vi "Visu acqui.vi"() -> ()   [LabVIEW 2022 SP3]
uses:
  Enum/Enum 7.ctl
  Variables globales/Variable glob generale.vi
  Variables globales/Variable globale compteurs.vi
  Variables globales/Variable glob Keller.vi
  Variables globales/Variable glob Pt.vi
  Variables globales/Variable glob Leybold.vi
  Variables globales/Variable glob Edwards.vi
  Variables globales/Variable glob Th.vi
  Variables globales/Variables glob EUROTHERM.vi
  Variables globales/Variable glob alertes pressions.vi
  Variables globales/Variable glob alertes min-max temperatures.vi
  Variables globales/Variable glob alertes ecart temperatures.vi
  Variables globales/Variable glob alertes Keller.vi
  Variables globales/Variable glob alertes Compteurs.vi
  <vilib>/Utility/config.llb/Write Key (String).vi
  <vilib>/Utility/config.llb/NI_LVConfig.lvlib
panel:
  in  "Y1/Y2":cluster{"Booléen":bool}[][](array[cluster]) caption="Y1    Y2"
  out "Alerte Compteurs":bool caption="Compteurs"
  in  "voir compteurs":bool caption="Valeurs compteurs"
  in  "Unités par":u16(ring) items=["seconde", "minute", "heure"]
  out "Pente":dbl format="%#.2g"
  in  "Capteur":u16(ring) items=[" keller1", "Compteur Sortie BLN2", "Débit Sortie BLN2"]
  in  "Calcul Pente":bool
  in  "voir alertes":bool caption="Définitions Alertes"
  out "nb capt":i32
  out "Noms visu":string[](array[string])
  out "Cuve":string
  out "Dossier distant":path
  out "référence en sortie":refnum<vi>
  out "SORTIE VISU":bool
  in  "Tout Y2":bool
  out "commentaire":string
  out "Dossier de sauvegarde":path
  in  "Tout Y1":bool
  in  "Tout OFF":bool
  out "Chemin du fichier local":path
  in  "Couleurs":u32[](array[colorbox])
  out "Alerte écart temp":bool caption="écarts températures"
  in  "Y2 log":bool caption="Y2 lin"
  in  "Y1 log":bool caption="Y1 lin"
  out "Alerte Keller":bool caption="Keller"
  out "Alerte min/max temp":bool caption="min/max températures"
  out "Données":string[](array[string])
  out "Alerte vide":bool caption="Vide"
  in  "grille Y2":bool
  in  "grille Y1":bool
  out "Courbe":cluster{dbl[], dbl[]}[](graph)
  in  "Echelles des Axes":bool=TRUE
  in  "SORTIR VISU":bool
  # "VISUALISATION ACQUISITIONS\ntempératures et pressions EN COURS"
  # "Ce logiciel et les informations qu'il contient, sont la propriété de l’IAS et ne peuvent être diffusés sans l’autorisation de la Station d’étalonnage"
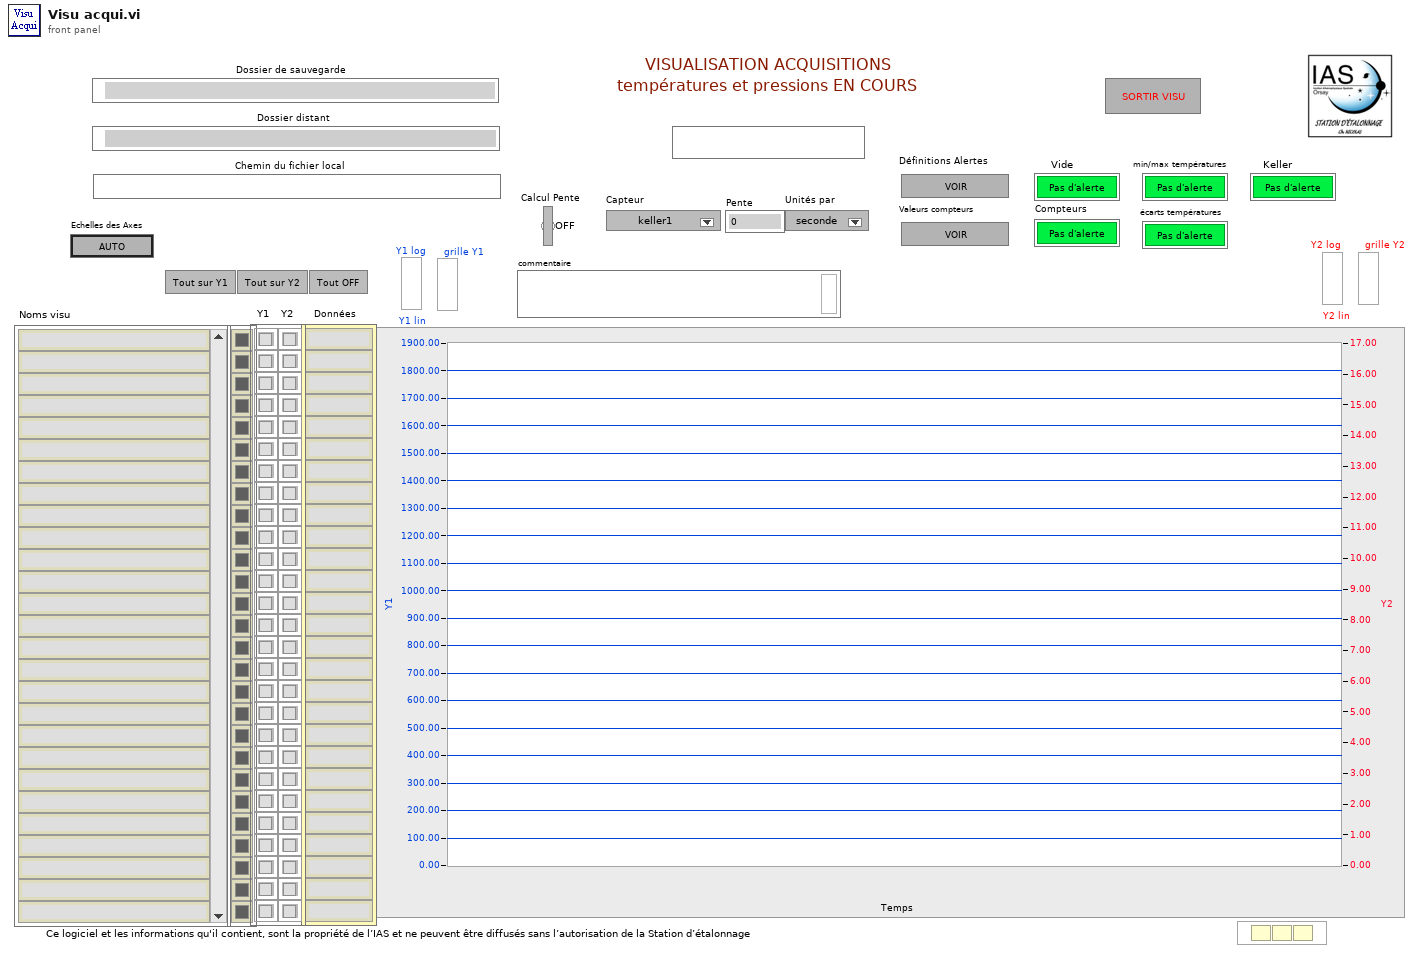
[diagram p1: front panel]
types:
  T1 = typedef "Enum 7.ctl" = enum16{"init", "choix", "init graph", "visu", "choix 2", "fin"}
  T2 = enum32{"Invalid", "Standard", "Closed", "Hidden", "Minimized", "Maximized"}
  T3 = cluster{"Noms voies select acqui 1COM":string[]}[]
  T4 = cluster{"Nom tache compteurs":refnum<k21>, "Noms des compteurs":string[], "Selection":bool[], "Init compteurs":dbl[], "Noms compteurs selectionnes":string[]}
  T5 = cluster{"Nom tache Pt":refnum<k21>, "Noms des Pt":string[], "Nb Pt":i16, "Selection Pt":bool[], "Nom Pt selectionnees":string[]}[]
  T6 = cluster{"Nom tache Th":refnum<k21>, "Noms des Th":string[], "Nb Th":i16, "Selection Th":bool[], "Nom Th selectionnes":string[]}[]
  T7 = cluster{"Alerte temp min/max":bool, "température max":dbl, "température min":dbl, "Défaut min/max temp":bool, "Indices à controler":i16[], "N°":u16}[]
  T8 = cluster{"Indices a controler":i16[], "Defaut":bool, "ecart temp":dbl, "Alerte":bool, ">?":bool, "N°":u16}[]
  T9 = cluster{"Alerte":bool, "valeur alerte":dbl, "Défaut":bool, "Indices à controler":i16[], "N°":u16}[]
  T10 = cluster{"Alerte":bool, "valeur ":dbl, "Défaut":bool, "Indices controler":i16[], "N°":u16}[]
  T11 = cluster{"Alerte Keller":bool, "valeur alerte Keller":dbl, "Défaut Keller":bool, "Indices Keller à controler":i16[], "N°":u16}[]
  T12 = typedef "NI_LVConfig.lvlib/Config Data RefNum.ctl" = refnum<k1>
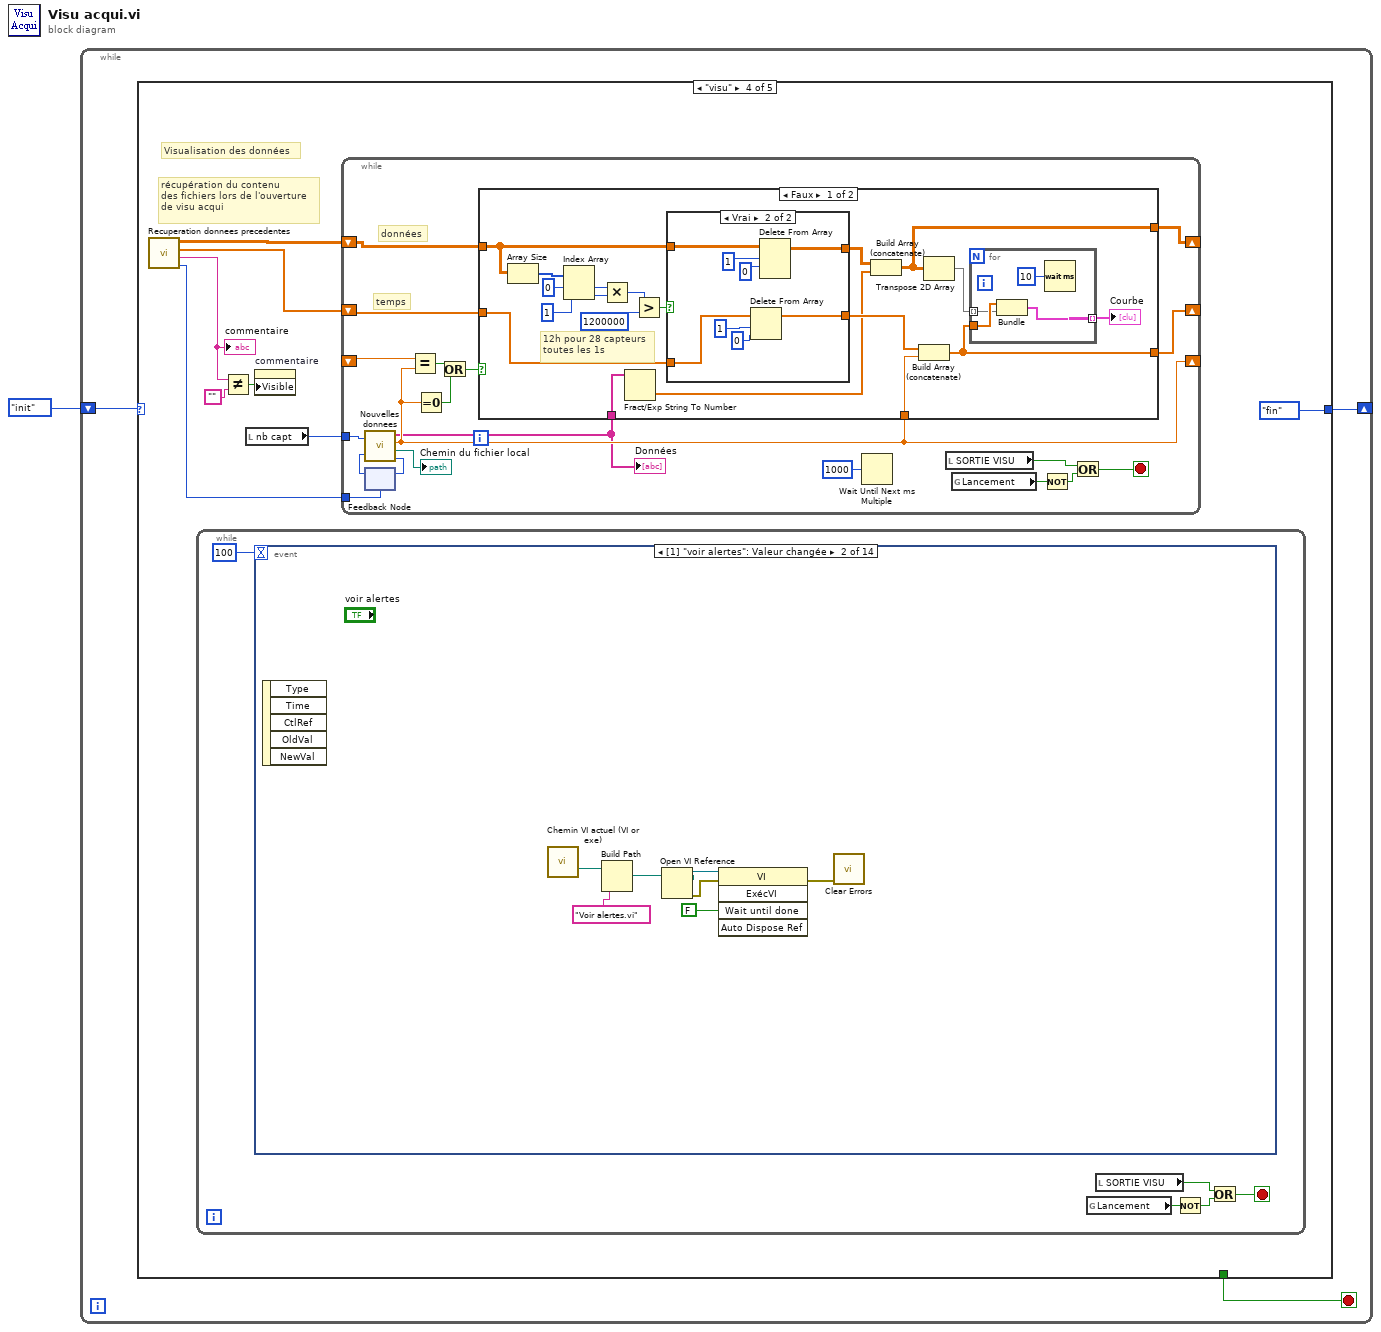
[diagram p0: block diagram]
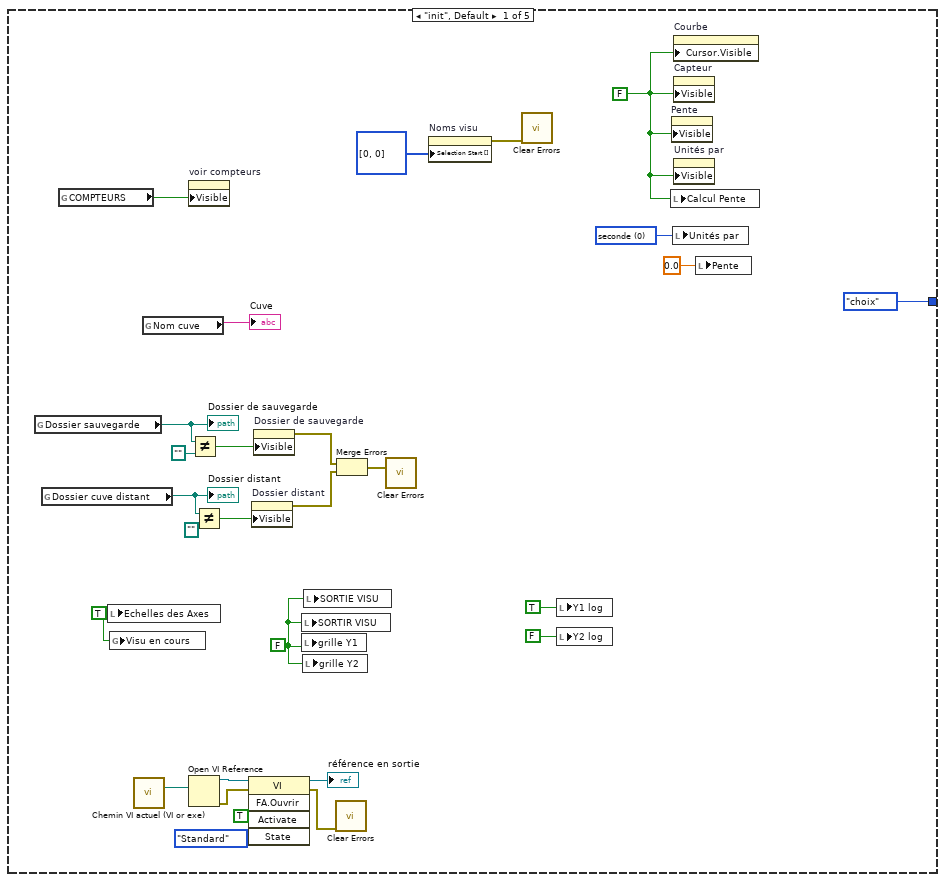
[diagram p2: hidden frame]
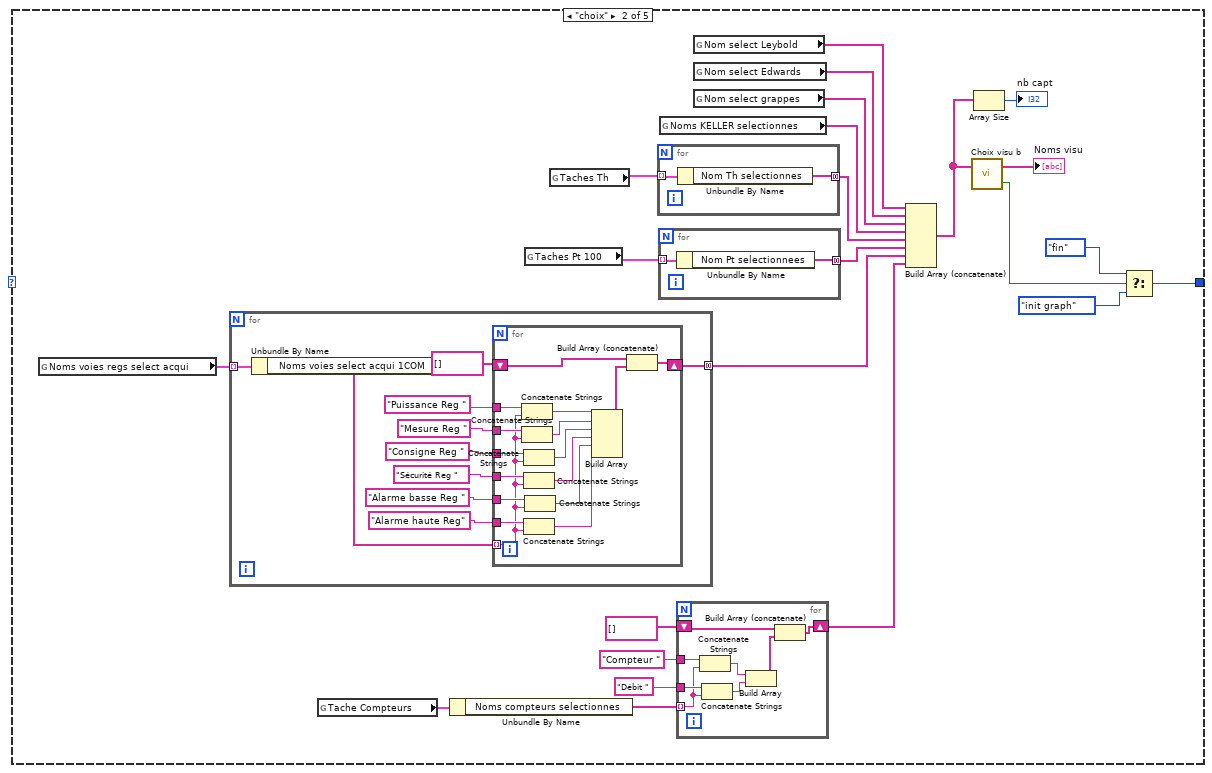
[diagram p3: hidden frame]
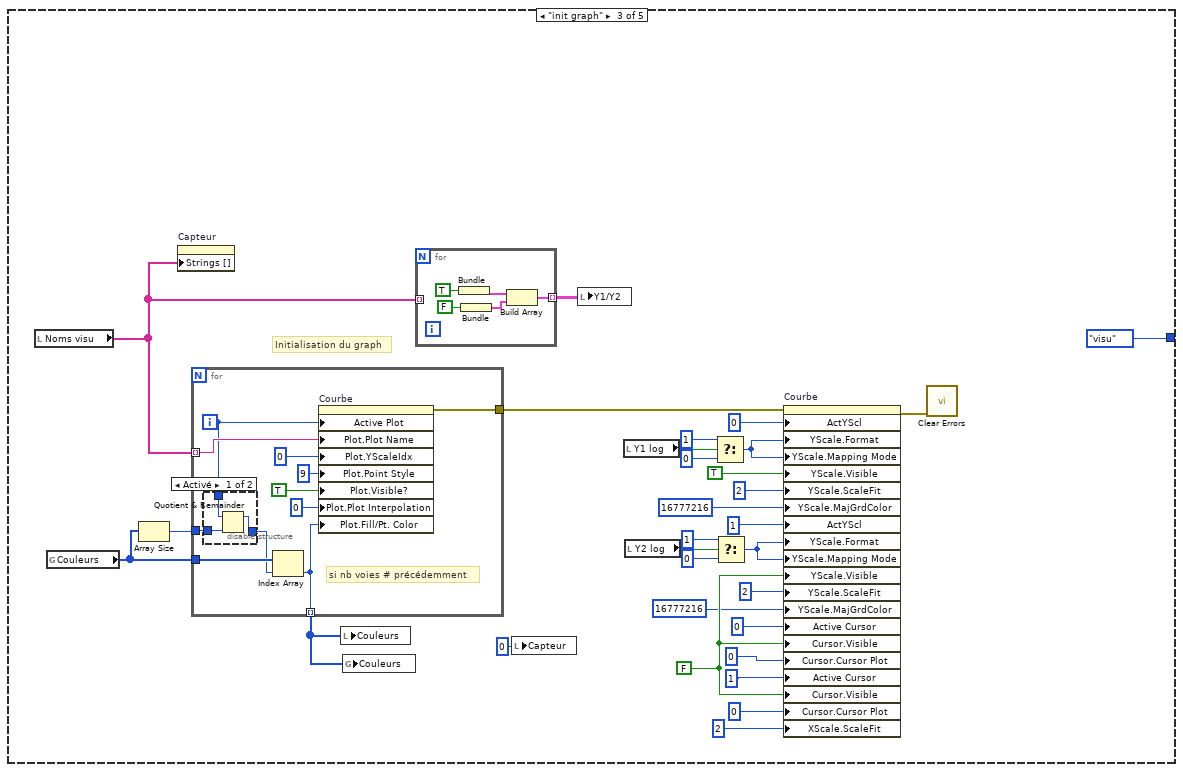
[diagram p4: hidden frame]
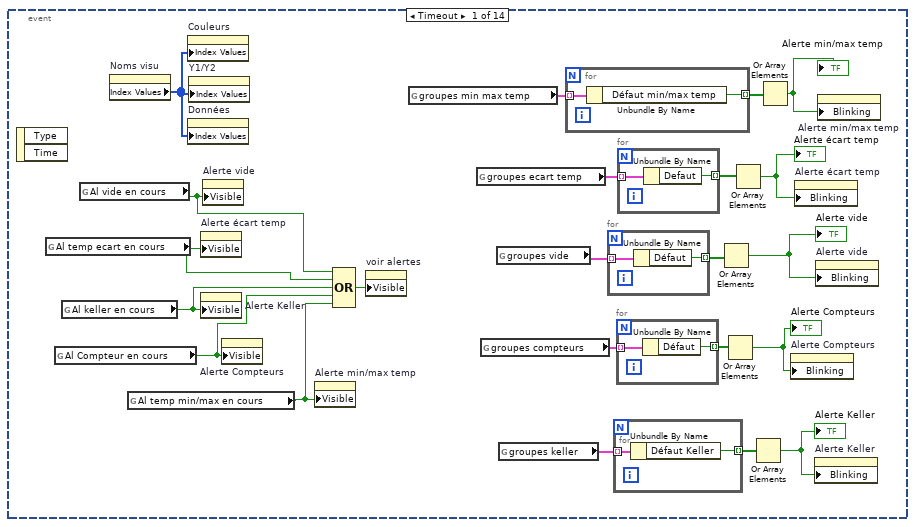
[diagram p6: hidden frame]
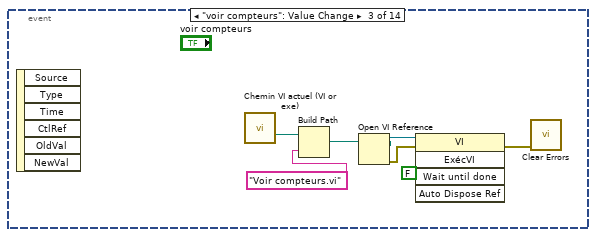
[diagram p7: hidden frame]
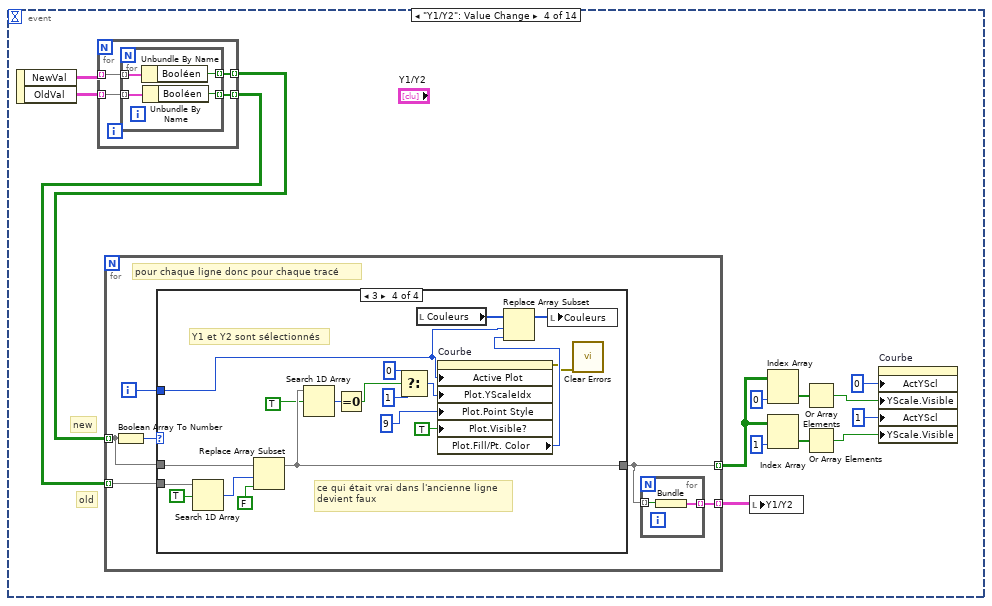
[diagram p8: hidden frame]
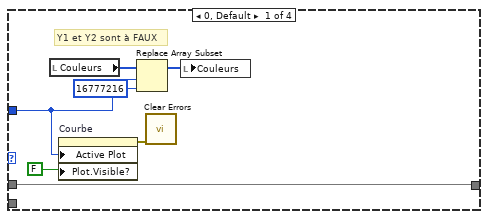
[diagram p9: hidden frame]
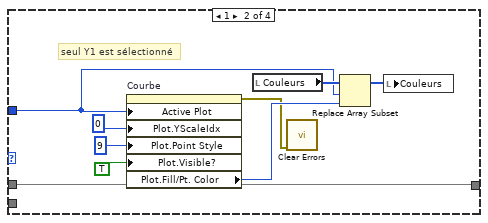
[diagram p10: hidden frame]
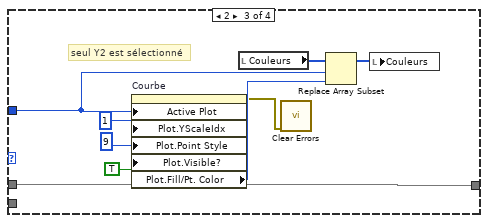
[diagram p11: hidden frame]
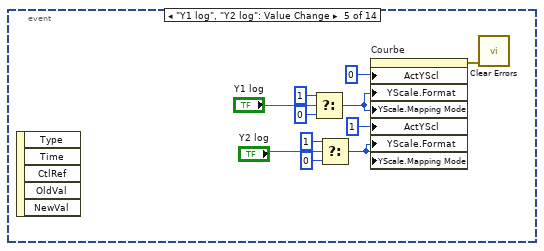
[diagram p12: hidden frame]
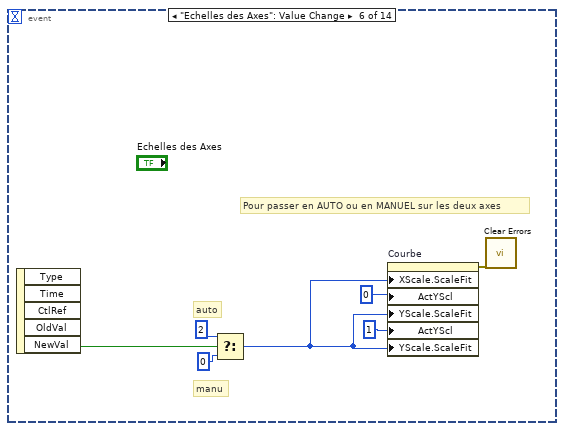
[diagram p13: hidden frame]
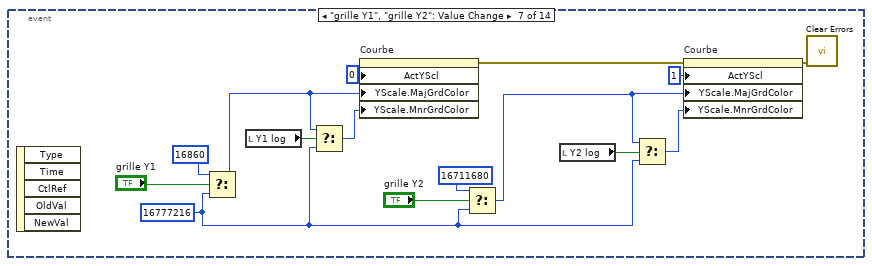
[diagram p14: hidden frame]
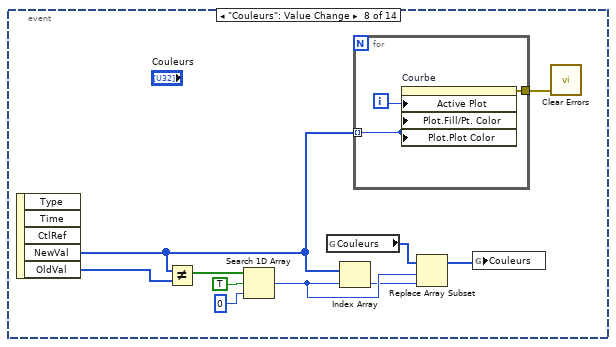
[diagram p15: hidden frame]
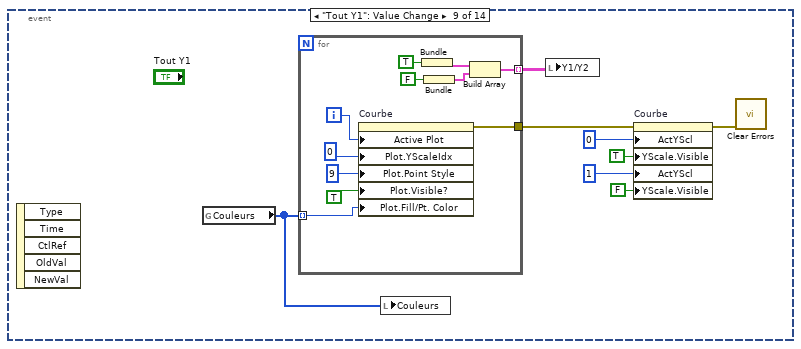
[diagram p16: hidden frame]
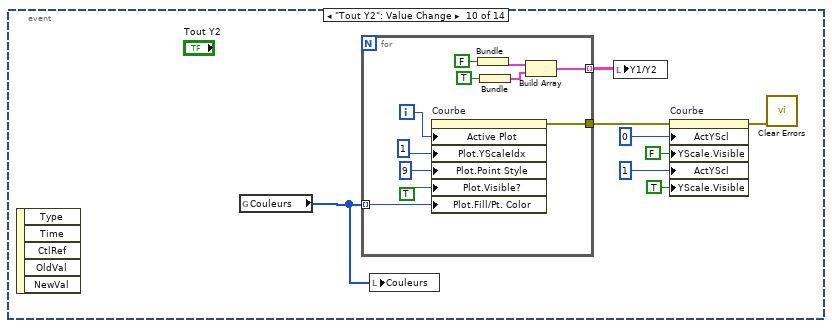
[diagram p17: hidden frame]
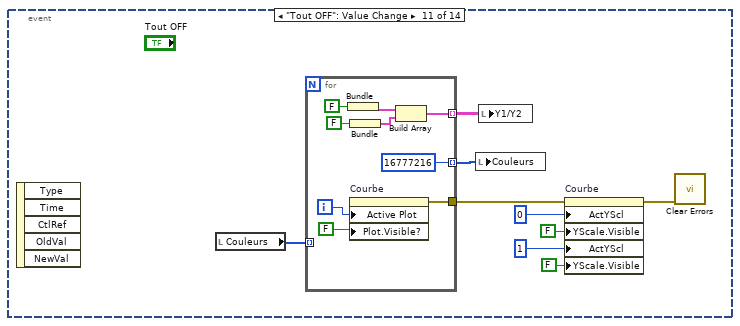
[diagram p18: hidden frame]
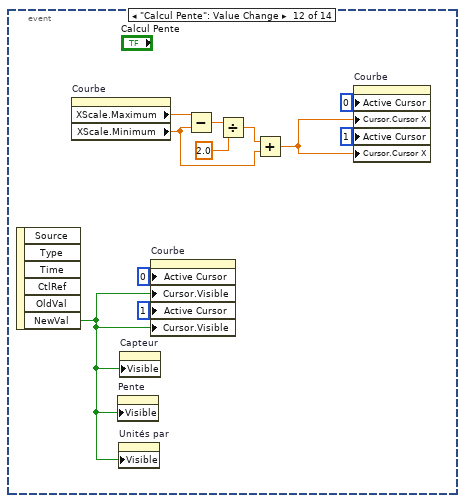
[diagram p19: hidden frame]
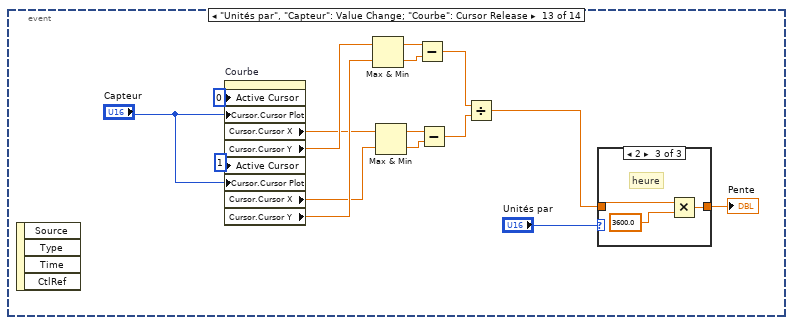
[diagram p20: hidden frame]
diagram:
  n1 = while {
    shift-right: [w3] -> _
    shift-left: Enum_7."init" ("Énum") -> [w4]
    stop <- w2 stop-if-true
    n2 = case shown="\"visu\"" w4 {
      tunnel: [Enum_7."choix" ("Énum") w46 Enum_7."visu" ("Énum") Enum_7."fin" ("Énum") Enum_7."init" ("Énum")] -> w3
      tunnel: [_ _ _ _ TRUE] -> w2
      frame "init", Default {
        w5 = u16 0 items=["seconde", "minute", "heure"] ("Unités par")
        w9 = FALSE
        w30 = TRUE ("Echelles des Axes")
        w31 = FALSE
        n3 = global read "Variable glob generale.vi" "Dossier sauvegarde"() -> (w29:path)
        "Dossier de sauvegarde" <- w29
        n4 = global read "Variable glob generale.vi" "Dossier cuve distant"() -> (w26:path)
        "Dossier distant" <- w26
        n5 = global read "Variable globale compteurs.vi" "COMPTEURS"() -> (w6:bool)
        n6 = local write "Echelles des Axes"(w30) -> ()
        n7 = global write "Variable glob generale.vi" "Visu en cours"(w30) -> ()
        n8 = call "Chemin VI actuel (VI or exe).vi"() -> ("Full Path to VI or executable"=w12:path)  [unwired: 14 in, 1 out]
        n9 = global read "Variable glob generale.vi" "Nom cuve"() -> (→"Cuve":string)
        n10 = property on="voir compteurs" class="Bool"("Visible"=w6) -> ()  [unwired: 2 in, 2 out]
        n11 = Open VI Reference(vi path=w12) -> (vi reference=w16:refnum<vi>, error out=w14:errorcluster)  [unwired: 5 in]
        n12 = Not Equal?(x=w29, y=path "") -> (x != y?=w27:bool)
        n13 = Not Equal?(x=w26, y=path "") -> (x != y?=w24:bool)
        n14 = invoke class="VI" method="FA.Ouvrir"(reference=w16, error in=w14, "Activate"=TRUE ("Activer ?"), "State"=T2."Standard" ("État")) -> (reference out=→"référence en sortie":refnum<vi>, error out=w13:errorcluster)  [unwired: 1 in, 3 out]
        n15 = property on="Dossier distant" class="Chm"("Visible"=w24) -> (error out=w21:errorcluster)  [unwired: 2 in, 1 out]
        n16 = property on="Dossier de sauvegarde" class="Chm"("Visible"=w27) -> (error out=w22:errorcluster)  [unwired: 2 in, 1 out]
        n17 = local write "SORTIR VISU"(w31) -> ()
        n18 = local write "grille Y1"(w31) -> ()
        n19 = local write "grille Y2"(w31) -> ()
        n20 = local write "SORTIE VISU"(w31) -> ()
        n21 = call <vilib>:"Clear Errors.vi"("error in (no error)"=w13) -> ()  [unwired: 5 in, 2 out]
        n22 = Merge Errors(w22, w21) -> (w23:errorcluster)
        n23 = call <vilib>:"Clear Errors.vi"("error in (no error)"=w23) -> ()  [unwired: 5 in, 2 out]
        n24 = property on="Noms visu" class="Tabl (strict)"("Selection Start []"=u32[] [0, 0] ("Début de sélection []")) -> (error out=w7:errorcluster)  [unwired: 2 in, 1 out]
        n25 = call <vilib>:"Clear Errors.vi"("error in (no error)"=w7) -> ()  [unwired: 5 in, 2 out]
        n26 = local write "Y1 log"(TRUE ("Y1 log")) -> ()
        n27 = local write "Y2 log"(FALSE ("Y2 log")) -> ()
        n28 = local write "Calcul Pente"(w9) -> ()
        n29 = property on="Pente" class="NumNb (strict)"("Visible"=w9) -> ()  [unwired: 2 in, 2 out]
        n30 = local write "Unités par"(w5) -> ()
        n31 = property on="Courbe" class="GraphXY (strict)"("Cursor.Visible"=w9) -> ()  [unwired: 2 in, 2 out]
        n32 = property on="Capteur" class="MDér (strict)"("Visible"=w9) -> ()  [unwired: 2 in, 2 out]
        n33 = property on="Unités par" class="MDér (strict)"("Visible"=w9) -> ()  [unwired: 2 in, 2 out]
        n34 = local write "Pente"(0.0 ("Pente")) -> ()
      }
      frame "choix" {
        n35 = global read "Variables glob EUROTHERM.vi" "Noms voies regs select acqui"() -> (w40:T3)
        n36 = for {
          tunnel: w40 -> [w73] mode=indexing
          tunnel: [w64] -> w39 mode=concatenating
          n37 = Unbundle By Name(w73) -> ("Noms voies select acqui 1COM"=w65:string[])
          n38 = for {
            tunnel: w65 -> [w83] mode=indexing
            tunnel: "Puissance Reg " -> [w89]
            tunnel: "Mesure Reg " -> [w88]
            tunnel: "Consigne Reg " -> [w87]
            tunnel: "Sécurité Reg " -> [w86]
            tunnel: "Alarme basse Reg " -> [w85]
            tunnel: "Alarme haute Reg" -> [w84]
            shift-right: [w74] -> w64
            shift-left: string[] [] -> [w75]
            n39 = Concatenate Strings(w89, w83) -> (w82:string)
            n40 = Concatenate Strings(w88, w83) -> (w81:string)
            n41 = Concatenate Strings(w87, w83) -> (w80:string)
            n42 = Concatenate Strings(w86, w83) -> (w79:string)
            n43 = Concatenate Strings(w84, w83) -> (w77:string)
            n44 = Concatenate Strings(w85, w83) -> (w78:string)
            n45 = Build Array(w82, w81, w80, w79, w78, w77) -> (w76:string[])
            n46 = Build Array (concatenate)(w75, w76) -> (w74:string[])
          }
        }
        n47 = global read "Variable globale compteurs.vi" "Tache Compteurs"() -> (w38:T4)
        n48 = Unbundle By Name(w38) -> ("Noms compteurs selectionnes"=w37:string[])
        n49 = global read "Variable glob Pt.vi" "Taches Pt 100"() -> (w44:T5)
        n50 = global read "Variable glob Th.vi" "Taches Th"() -> (w42:T6)
        n51 = for {
          tunnel: w42 -> [w91] mode=indexing
          tunnel: [w90] -> w41 mode=concatenating
          n52 = Unbundle By Name(w91) -> ("Nom Th selectionnes"=w90:string[])
        }
        n53 = for {
          tunnel: w44 -> [w93] mode=indexing
          tunnel: [w92] -> w43 mode=concatenating
          n54 = Unbundle By Name(w93) -> ("Nom Pt selectionnees"=w92:string[])
        }
        n55 = global read "Variable glob Keller.vi" "Noms KELLER selectionnes"() -> (w53:string[])
        n56 = for {
          tunnel: w37 -> [w61] mode=indexing
          tunnel: "Compteur " -> [w63]
          tunnel: "Débit " -> [w62]
          shift-right: [w57] -> w33
          shift-left: string[] [] -> [w58]
          n57 = Concatenate Strings(w63, w61) -> (w60:string)
          n58 = Concatenate Strings(w62, w61) -> (w59:string)
          n59 = Build Array(w60, w59) -> (w56:string[])
          n60 = Build Array (concatenate)(w58, w56) -> (w57:string[])
        }
        n61 = global read "Variable glob Leybold.vi" "Nom select Leybold"() -> (w54:string[])
        n62 = global read "Variable glob Edwards.vi" "Nom select Edwards"() -> (w55:string[])
        n63 = global read "Variable glob Edwards.vi" "Nom select grappes"() -> (w45:string[])
        n64 = Build Array (concatenate)(w54, w55, w45, w53, w41, w43, w39, w33) -> (w50:string[])
        n65 = call "Choix visu b.vi"("Noms"=w50) -> ("annulé"=w49:bool, "Noms 2"=→"Noms visu":string[])  [unwired: 1 in]
        n66 = Array Size(array=w50) -> (size(s)=→"nb capt":i32)
        n67 = Select(t=Enum_7."fin" ("Énum"), s=w49, f=Enum_7."init graph" ("Énum")) -> (s? t:f=w46:T1)
      }
      frame "init graph" {
        w104 = FALSE ("Échelle des Y.Visible")
        # "Initialisation du graph"
        n68 = local read "Noms visu"() -> (w95:string[])
        n69 = global read "Variable glob generale.vi" "Couleurs"() -> (w123:u32[])
        n70 = Array Size(array=w123) -> (size(s)=w122:i32)
        n71 = property on="Capteur" class="MDér (strict)"("Strings []"=w95) -> ()  [unwired: 2 in, 2 out]
        n72 = for {
          tunnel: w95 -> [w139] mode=indexing
          tunnel: [w133] -> w121 mode=indexing
          tunnel: w123 -> [w134]
          tunnel: w122 -> [w131]
          tunnel: [w130] -> w119
          i -> [w129]
          # "si nb voies # précédemment"
          n73 = disable-structure shown="Activé" {
            disable-tunnel: [w142 w143] -> w132
            disable-tunnel: w131 -> [w141 _]
            disable-tunnel: w129 -> [w140 w143]
            frame Enabled {
              n74 = Quotient & Remainder(x=w140, y=w141) -> (x-y*floor(x/y)=w142:i32)  [unwired: 1 out]
            }
            frame Disabled {
            }
          }
          n75 = Index Array(array=w134, index=w132) -> (element=w133:u32)
          n76 = property on="Courbe" class="GraphXY (strict)"("Active Plot"=w129, "Plot.Plot Name"=w139, "Plot.YScaleIdx"=u32 0 ("Tracé.Indice d'échelle des Y"), "Plot.Point Style"=u8 9 ("Tracé.Style de point"), "Plot.Visible?"=TRUE, "Plot.Plot Interpolation"=u32 0 ("Tracé.Indice d'échelle des Y"), "Plot.Fill/Pt. Color"=w133) -> (error out=w130:errorcluster)  [unwired: 2 in, 1 out]
        }
        n77 = local write "Couleurs"(w121) -> ()
        n78 = global write "Variable glob generale.vi" "Couleurs"(w121) -> ()
        n79 = for {
          tunnel: w95 -> [_] mode=indexing
          tunnel: [w124] -> w94 mode=indexing
          n80 = Bundle(TRUE) -> (w126:cluster{bool})  [unwired: 1 in]
          n81 = Bundle(FALSE) -> (w125:cluster{bool})  [unwired: 1 in]
          n82 = Build Array(w126, w125) -> (w124:cluster{bool}[])
        }
        n83 = local write "Capteur"(u16 0) -> ()
        n84 = local write "Y1/Y2"(w94) -> ()
        n85 = local read "Y1 log"() -> (w111:bool)
        n86 = local read "Y2 log"() -> (w110:bool)
        n87 = Select(t=u8 1 ("cas vrai"), s=w111, f=u8 0 ("cas faux")) -> (s? t:f=w112:u8)
        n88 = Select(t=u8 1 ("cas vrai"), s=w110, f=u8 0 ("cas faux")) -> (s? t:f=w108:u8)
        n89 = property on="Courbe" class="GraphXY (strict)"(error in=w119, "ActYScl"=0 ("Échelle active des Y"), "YScale.Format"=w112, "YScale.Mapping Mode"=w112, "YScale.Visible"=TRUE ("Échelle des Y.Visible"), "YScale.ScaleFit"=u8 2 ("Échelle des X.Ajuster l'échelle"), "YScale.MajGrdColor"=u32 16777216 ("cas faux"), "ActYScl"=1 ("Échelle active des Y"), "YScale.Format"=w108, "YScale.Mapping Mode"=w108, "YScale.Visible"=w104, "YScale.ScaleFit"=u8 2 ("Échelle des X.Ajuster l'échelle"), "YScale.MajGrdColor"=u32 16777216 ("cas faux"), "Active Cursor"=u32 0 ("Curseur actif"), "Cursor.Visible"=w104, "Cursor.Cursor Plot"=0 ("Curseur.Tracé du curseur"), "Active Cursor"=u32 1 ("Curseur actif"), "Cursor.Visible"=w104, "Cursor.Cursor Plot"=0 ("Curseur.Tracé du curseur"), "XScale.ScaleFit"=u8 2 ("Échelle des X.Ajuster l'échelle")) -> (error out=w118:errorcluster)  [unwired: 1 in, 1 out]
        n90 = call <vilib>:"Clear Errors.vi"("error in (no error)"=w118) -> ()  [unwired: 5 in, 2 out]
      }
      frame "visu" {
        # "récupération du contenu\ndes fichiers lors de l'ouverture\nde visu acqui"
        # "Visualisation des données"
        n91 = call "Recuperation donnees precedentes.vi"() -> ("Données"=w151:dbl[][], "Temps"=w150:dbl[], "commentaire"=w149:string, "offset (en octets)"=w146:i64)  [unwired: 2 in]
        "commentaire" <- w149
        n92 = while {
          stop <- w155 stop-if-true
          n93 = event shown="[1] \"voir alertes\": Valeur changée" {
            selector: _ -> [_ _ _ _ _ _ _ _ _ _ _ _ _ _]
            dyn-events: _ -> [_ _ _ _ _ _ _ _ _ _ _ _ _ _]
            timeout: 100 -> [_ _ _ _ _ _ _ _ _ _ _ _ _ _]
            event Timeout {
              n94 = event-data() -> ()  [unwired: 1 in, 2 out]
              n95 = global read "Variable glob alertes ecart temperatures.vi" "Al temp ecart en cours"() -> (w175:bool)
              n96 = global read "Variable glob alertes Compteurs.vi" "Al Compteur en cours"() -> (w172:bool)
              n97 = global read "Variable glob alertes Keller.vi" "Al keller en cours"() -> (w174:bool)
              n98 = global read "Variable glob alertes pressions.vi" "Al vide en cours"() -> (w176:bool)
              n99 = property on="Noms visu" class="Tabl (strict)"() -> ("Index Values"=w178:u32[])  [unwired: 2 in, 2 out]
              n100 = global read "Variable glob alertes min-max temperatures.vi" "Al temp min/max en cours"() -> (w173:bool)
              n101 = property on="Couleurs" class="Tabl (strict)"("Index Values"=w178) -> ()  [unwired: 2 in, 2 out]
              n102 = property on="Données" class="Tabl (strict)"("Index Values"=w178) -> ()  [unwired: 2 in, 2 out]
              n103 = property on="Y1/Y2" class="Tabl (strict)"("Index Values"=w178) -> ()  [unwired: 2 in, 2 out]
              n104 = property on="Alerte écart temp" class="Bool (strict)"("Visible"=w175) -> ()  [unwired: 2 in, 2 out]
              n105 = property on="Alerte Keller" class="Bool (strict)"("Visible"=w174) -> ()  [unwired: 2 in, 2 out]
              n106 = property on="Alerte vide" class="Bool (strict)"("Visible"=w176) -> ()  [unwired: 2 in, 2 out]
              n107 = property on="Alerte Compteurs" class="Bool (strict)"("Visible"=w172) -> ()  [unwired: 2 in, 2 out]
              n108 = property on="Alerte min/max temp" class="Bool (strict)"("Visible"=w173) -> ()  [unwired: 2 in, 2 out]
              n109 = Compound Arithmetic op=OR(w176, w175, w174, w172, w173) -> (w177:bool)
              n110 = property on="voir alertes" class="Bool"("Visible"=w177) -> ()  [unwired: 2 in, 2 out]
              n111 = global read "Variable glob alertes min-max temperatures.vi" "groupes min max temp"() -> (w168:T7)
              n112 = global read "Variable glob alertes ecart temperatures.vi" "groupes ecart temp"() -> (w171:T8)
              n113 = global read "Variable glob alertes Compteurs.vi" "groupes compteurs"() -> (w159:T9)
              n114 = global read "Variable glob alertes pressions.vi" "groupes vide"() -> (w162:T10)
              n115 = global read "Variable glob alertes Keller.vi" "groupes keller"() -> (w165:T11)
              n116 = for {
                tunnel: w168 -> [w186] mode=indexing
                tunnel: [w185] -> w167 mode=indexing
                n117 = Unbundle By Name(w186) -> ("Défaut min/max temp"=w185:bool)
              }
              n118 = for {
                tunnel: w162 -> [w182] mode=indexing
                tunnel: [w181] -> w161 mode=indexing
                n119 = Unbundle By Name(w182) -> ("Défaut"=w181:bool)
              }
              n120 = for {
                tunnel: w165 -> [w184] mode=indexing
                tunnel: [w183] -> w164 mode=indexing
                n121 = Unbundle By Name(w184) -> ("Défaut Keller"=w183:bool)
              }
              n122 = for {
                tunnel: w159 -> [w180] mode=indexing
                tunnel: [w179] -> w158 mode=indexing
                n123 = Unbundle By Name(w180) -> ("Défaut"=w179:bool)
              }
              n124 = for {
                tunnel: w171 -> [w188] mode=indexing
                tunnel: [w187] -> w170 mode=indexing
                n125 = Unbundle By Name(w188) -> ("Defaut"=w187:bool)
              }
              n126 = Or Array Elements(Boolean array=w161) -> (logical OR=w160:bool)
              "Alerte vide" <- w160
              n127 = Or Array Elements(Boolean array=w158) -> (logical OR=w157:bool)
              "Alerte Compteurs" <- w157
              n128 = Or Array Elements(Boolean array=w170) -> (logical OR=w169:bool)
              "Alerte écart temp" <- w169
              n129 = Or Array Elements(Boolean array=w164) -> (logical OR=w163:bool)
              "Alerte Keller" <- w163
              n130 = Or Array Elements(Boolean array=w167) -> (logical OR=w166:bool)
              "Alerte min/max temp" <- w166
              n131 = property on="Alerte Compteurs" class="Bool (strict)"("Blinking"=w157) -> ()  [unwired: 2 in, 2 out]
              n132 = property on="Alerte écart temp" class="Bool (strict)"("Blinking"=w169) -> ()  [unwired: 2 in, 2 out]
              n133 = property on="Alerte Keller" class="Bool (strict)"("Blinking"=w163) -> ()  [unwired: 2 in, 2 out]
              n134 = property on="Alerte vide" class="Bool (strict)"("Blinking"=w160) -> ()  [unwired: 2 in, 2 out]
              n135 = property on="Alerte min/max temp" class="Bool (strict)"("Blinking"=w166) -> ()  [unwired: 2 in, 2 out]
            }
            event "voir alertes": Value Change {
              n136 = event-data() -> ()  [unwired: 1 in, 5 out]
              n137 = call "Chemin VI actuel (VI or exe).vi"() -> ("VI or executable installation directory"=w189:path)  [unwired: 14 in, 1 out]
              n138 = Build Path(base path=w189, name or relative path="Voir alertes.vi" ("nom ou chemin relatif")) -> (appended path=w194:path)
              n139 = Open VI Reference(vi path=w194) -> (vi reference=w192:refnum<vi>, error out=w191:errorcluster)  [unwired: 5 in]
              n140 = invoke class="VI" method="ExécVI"(reference=w192, error in=w191, "Wait until done"=FALSE ("Attendre la fin")) -> (error out=w190:errorcluster)  [unwired: 2 in, 4 out]
              n141 = call <vilib>:"Clear Errors.vi"("error in (no error)"=w190) -> ()  [unwired: 5 in, 2 out]
            }
            event "voir compteurs": Value Change {
              n142 = event-data() -> ()  [unwired: 1 in, 6 out]
              n143 = call "Chemin VI actuel (VI or exe).vi"() -> ("VI or executable installation directory"=w198:path)  [unwired: 14 in, 1 out]
              n144 = Build Path(base path=w198, name or relative path="Voir compteurs.vi" ("nom ou chemin relatif")) -> (appended path=w202:path)
              n145 = Open VI Reference(vi path=w202) -> (vi reference=w201:refnum<vi>, error out=w200:errorcluster)  [unwired: 5 in]
              n146 = invoke class="VI" method="ExécVI"(reference=w201, error in=w200, "Wait until done"=FALSE ("Attendre la fin")) -> (error out=w199:errorcluster)  [unwired: 2 in, 4 out]
              n147 = call <vilib>:"Clear Errors.vi"("error in (no error)"=w199) -> ()  [unwired: 5 in, 2 out]
            }
            event "Y1/Y2": Value Change {
              # "old"
              # "new"
              n148 = event-data() -> ("NewVal"=w207:cluster{"Booléen":bool}[][], "OldVal"=w206:cluster{"Booléen":bool}[][])  [unwired: 1 in]
              n149 = for {
                tunnel: w207 -> [w220] mode=indexing
                tunnel: [w219] -> w205 mode=indexing
                tunnel: w206 -> [w218] mode=indexing
                tunnel: [w217] -> w204 mode=indexing
                n150 = for {
                  tunnel: w220 -> [w224] mode=indexing
                  tunnel: [w223] -> w219 mode=indexing
                  tunnel: [w222] -> w217 mode=indexing
                  tunnel: w218 -> [w221] mode=indexing
                  n151 = Unbundle By Name(w224) -> ("Booléen"=w223:bool)
                  n152 = Unbundle By Name(w221) -> ("Booléen"=w222:bool)
                }
              }
              n153 = for {
                tunnel: w205 -> [w227] mode=indexing
                tunnel: w204 -> [w228] mode=indexing
                tunnel: [w226] -> w210 mode=indexing
                tunnel: [w225] -> w203 mode=indexing
                i -> [w230]
                # "pour chaque ligne donc pour chaque tracé"
                n154 = Boolean Array To Number(Boolean array=w227) -> (number=w229:u32)
                n155 = case shown="3" w229 {
                  tunnel: w230 -> [w236 w242 w250 w260]
                  tunnel: w228 -> [_ _ _ w273]
                  tunnel: [w238 w246 w255 w268] -> w226
                  tunnel: w227 -> [w238 w246 w255 w269]
                  frame 0, Default {
                    # "Y1 et Y2 sont à FAUX"
                    n156 = local read "Couleurs"() -> (w237:u32[])
                    n157 = property on="Courbe" class="GraphXY (strict)"("Active Plot"=w236, "Plot.Visible?"=FALSE) -> (error out=w233:errorcluster)  [unwired: 2 in, 1 out]
                    n158 = Replace Array Subset(array=w237, new element=u32 16777216 ("nouvel élément/sous-tableau"), index=w236) -> (w235:u32[])
                    n159 = call <vilib>:"Clear Errors.vi"("error in (no error)"=w233) -> ()  [unwired: 5 in, 2 out]
                    n160 = local write "Couleurs"(w235) -> ()
                  }
                  frame 1 {
                    # "seul Y1 est sélectionné"
                    n161 = property on="Courbe" class="GraphXY (strict)"("Active Plot"=w242, "Plot.YScaleIdx"=i8 0 ("cas faux"), "Plot.Point Style"=i8 9 ("cas faux"), "Plot.Visible?"=TRUE) -> (error out=w240:errorcluster, "Plot.Fill/Pt. Color"=w241:u32)  [unwired: 2 in, 1 out]
                    n162 = local read "Couleurs"() -> (w244:u32[])
                    n163 = call <vilib>:"Clear Errors.vi"("error in (no error)"=w240) -> ()  [unwired: 5 in, 2 out]
                    n164 = Replace Array Subset(array=w244, new element=w241, index=w242) -> (w243:u32[])
                    n165 = local write "Couleurs"(w243) -> ()
                  }
                  frame 2 {
                    # "seul Y2 est sélectionné"
                    n166 = property on="Courbe" class="GraphXY (strict)"("Active Plot"=w250, "Plot.YScaleIdx"=i8 1 ("cas vrai"), "Plot.Point Style"=i8 9 ("cas vrai"), "Plot.Visible?"=TRUE) -> (error out=w249:errorcluster, "Plot.Fill/Pt. Color"=w251:u32)  [unwired: 2 in, 1 out]
                    n167 = local read "Couleurs"() -> (w253:u32[])
                    n168 = call <vilib>:"Clear Errors.vi"("error in (no error)"=w249) -> ()  [unwired: 5 in, 2 out]
                    n169 = Replace Array Subset(array=w253, new element=w251, index=w250) -> (w252:u32[])
                    n170 = local write "Couleurs"(w252) -> ()
                  }
                  frame 3 {
                    # "ce qui était vrai dans l'ancienne ligne\ndevient faux"
                    # "Y1 et Y2 sont sélectionnés"
                    n171 = Search 1D Array(1D array=w273, element=TRUE) -> (index of element=w275:i32)  [unwired: 1 in]
                    n172 = Replace Array Subset(array=w269, new element=FALSE, index=w275) -> (w268:bool[])
                    n173 = Search 1D Array(1D array=w268, element=TRUE) -> (index of element=w266:i32)  [unwired: 1 in]
                    n174 = Equal To 0?(x=w266) -> (x = 0?=w265:bool)
                    n175 = Select(t=i8 0 ("cas vrai"), s=w265, f=i8 1 ("cas faux")) -> (s? t:f=w272:i8)
                    n176 = local read "Couleurs"() -> (w263:u32[])
                    n177 = property on="Courbe" class="GraphXY (strict)"("Active Plot"=w260, "Plot.YScaleIdx"=w272, "Plot.Point Style"=i8 9 ("cas vrai"), "Plot.Visible?"=TRUE) -> (error out=w258:errorcluster, "Plot.Fill/Pt. Color"=w261:u32)  [unwired: 2 in, 1 out]
                    n178 = Replace Array Subset(array=w263, new element=w261, index=w260) -> (w262:u32[])
                    n179 = local write "Couleurs"(w262) -> ()
                    n180 = call <vilib>:"Clear Errors.vi"("error in (no error)"=w258) -> ()  [unwired: 5 in, 2 out]
                  }
                }
                n181 = for {
                  tunnel: w226 -> [w232] mode=indexing
                  tunnel: [w231] -> w225 mode=indexing
                  n182 = Bundle("Booléen"=w232) -> (w231:cluster{"Booléen":bool})  [unwired: 1 in]
                }
              }
              n183 = local write "Y1/Y2"(w203) -> ()
              n184 = Index Array(array=w210, index (col)=0 ("indice désactivé (col)")) -> (element=w213:bool[])  [unwired: 1 in]
              n185 = Index Array(array=w210, index (col)=1 ("indice désactivé (col)")) -> (element=w212:bool[])  [unwired: 1 in]
              n186 = Or Array Elements(Boolean array=w213) -> (logical OR=w209:bool)
              n187 = Or Array Elements(Boolean array=w212) -> (logical OR=w208:bool)
              n188 = property on="Courbe" class="GraphXY (strict)"("ActYScl"=0 ("Échelle active des Y"), "YScale.Visible"=w209, "ActYScl"=1 ("Échelle active des Y"), "YScale.Visible"=w208) -> ()  [unwired: 2 in, 2 out]
            }
            event "Y1 log", "Y2 log": Value Change {
              n189 = event-data() -> ()  [unwired: 1 in, 5 out]
              n190 = Select(t=i8 1 ("cas vrai"), s="Y1 log", f=i8 0 ("cas faux")) -> (s? t:f=w283:i8)
              n191 = Select(t=i8 1 ("cas vrai"), s="Y2 log", f=i8 0 ("cas faux")) -> (s? t:f=w286:i8)
              n192 = property on="Courbe" class="GraphXY (strict)"("ActYScl"=0 ("Échelle active des Y"), "YScale.Format"=w283, "YScale.Mapping Mode"=w283, "ActYScl"=1 ("Échelle active des Y"), "YScale.Format"=w286, "YScale.Mapping Mode"=w286) -> (error out=w277:errorcluster)  [unwired: 2 in, 1 out]
              n193 = call <vilib>:"Clear Errors.vi"("error in (no error)"=w277) -> ()  [unwired: 5 in, 2 out]
            }
            event "Echelles des Axes": Value Change {
              # "manu"
              # "auto"
              # "Pour passer en AUTO ou en MANUEL sur les deux axes"
              n194 = event-data() -> ("NewVal"=w292:bool)  [unwired: 1 in, 4 out]
              n195 = Select(t=u8 2 ("cas vrai"), s=w292, f=u8 0 ("Échelle des X.Ajuster l'échelle")) -> (s? t:f=w290:u8)
              n196 = property on="Courbe" class="GraphXY (strict)"("XScale.ScaleFit"=w290, "ActYScl"=0, "YScale.ScaleFit"=w290, "ActYScl"=1, "YScale.ScaleFit"=w290) -> (error out=w288:errorcluster)  [unwired: 2 in, 1 out]
              n197 = call <vilib>:"Clear Errors.vi"("error in (no error)"=w288) -> ()  [unwired: 5 in, 2 out]
            }
            event "grille Y1", "grille Y2": Value Change {
              w295 = 16777216 ("cas faux")
              n198 = event-data() -> ()  [unwired: 1 in, 5 out]
              n199 = Select(t=16860 ("cas vrai"), s="grille Y1", f=w295) -> (s? t:f=w299:i32)
              n200 = local read "Y1 log"() -> (w301:bool)
              n201 = Select(t=w299, s=w301, f=w295) -> (s? t:f=w300:i32)
              n202 = property on="Courbe" class="GraphXY (strict)"("ActYScl"=0 ("Échelle active des Y"), "YScale.MajGrdColor"=w299, "YScale.MnrGrdColor"=w300) -> (error out=w308:errorcluster)  [unwired: 2 in, 1 out]
              n203 = Select(t=16711680 ("cas vrai"), s="grille Y2", f=w295) -> (s? t:f=w297:i32)
              n204 = local read "Y2 log"() -> (w298:bool)
              n205 = Select(t=w297, s=w298, f=w295) -> (s? t:f=w296:i32)
              n206 = property on="Courbe" class="GraphXY (strict)"(error in=w308, "ActYScl"=1 ("Échelle active des Y"), "YScale.MajGrdColor"=w297, "YScale.MnrGrdColor"=w296) -> (error out=w302:errorcluster)  [unwired: 1 in, 1 out]
              n207 = call <vilib>:"Clear Errors.vi"("error in (no error)"=w302) -> ()  [unwired: 5 in, 2 out]
            }
            event "Couleurs": Value Change {
              n208 = event-data() -> ("NewVal"=w315:u32[], "OldVal"=w319:u32[])  [unwired: 1 in, 3 out]
              n209 = Not Equal?(x=w315, y=w319) -> (x != y?=w318:bool[])
              n210 = Search 1D Array(1D array=w318, element=TRUE ("élément"), start index (0)=0 ("indice de départ (0)")) -> (index of element=w313:i32)
              n211 = global read "Variable glob generale.vi" "Couleurs"() -> (w314:u32[])
              n212 = Index Array(array=w315, index=w313) -> (element=w312:u32)
              n213 = for {
                tunnel: w315 -> [w321] mode=indexing
                tunnel: [w320] -> w310
                i -> [w322]
                n214 = property on="Courbe" class="GraphXY (strict)"("Active Plot"=w322, "Plot.Fill/Pt. Color"=w321, "Plot.Plot Color"=w321) -> (error out=w320:errorcluster)  [unwired: 2 in, 1 out]
              }
              n215 = Replace Array Subset(array=w314, new element=w312, index=w313) -> (w311:u32[])
              n216 = global write "Variable glob generale.vi" "Couleurs"(w311) -> ()
              n217 = call <vilib>:"Clear Errors.vi"("error in (no error)"=w310) -> ()  [unwired: 5 in, 2 out]
            }
            event "Tout Y1": Value Change {
              n218 = event-data() -> ()  [unwired: 1 in, 5 out]
              n219 = global read "Variable glob generale.vi" "Couleurs"() -> (w330:u32[])
              n220 = for {
                tunnel: w330 -> [w337] mode=indexing
                tunnel: [w336] -> w325
                tunnel: [w331] -> w323 mode=indexing
                i -> [w338]
                n221 = property on="Courbe" class="GraphXY (strict)"("Active Plot"=w338, "Plot.YScaleIdx"=i8 0 ("cas faux"), "Plot.Point Style"=i8 9 ("cas faux"), "Plot.Visible?"=TRUE, "Plot.Fill/Pt. Color"=w337) -> (error out=w336:errorcluster)  [unwired: 2 in, 1 out]
                n222 = Bundle(TRUE) -> (w334:cluster{bool})  [unwired: 1 in]
                n223 = Bundle(FALSE) -> (w335:cluster{bool})  [unwired: 1 in]
                n224 = Build Array(w334, w335) -> (w331:cluster{bool}[])
              }
              n225 = local write "Couleurs"(w330) -> ()
              n226 = local write "Y1/Y2"(w323) -> ()
              n227 = property on="Courbe" class="GraphXY (strict)"(error in=w325, "ActYScl"=0 ("Échelle active des Y"), "YScale.Visible"=TRUE ("Échelle des Y.Visible"), "ActYScl"=1 ("Échelle active des Y"), "YScale.Visible"=FALSE ("Échelle des Y.Visible")) -> (error out=w324:errorcluster)  [unwired: 1 in, 1 out]
              n228 = call <vilib>:"Clear Errors.vi"("error in (no error)"=w324) -> ()  [unwired: 5 in, 2 out]
            }
            event "Tout Y2": Value Change {
              n229 = event-data() -> ()  [unwired: 1 in, 5 out]
              n230 = global read "Variable glob generale.vi" "Couleurs"() -> (w349:u32[])
              n231 = for {
                tunnel: w349 -> [w356] mode=indexing
                tunnel: [w355] -> w344
                tunnel: [w350] -> w342 mode=indexing
                i -> [w357]
                n232 = property on="Courbe" class="GraphXY (strict)"("Active Plot"=w357, "Plot.YScaleIdx"=i8 1 ("cas faux"), "Plot.Point Style"=i8 9 ("cas faux"), "Plot.Visible?"=TRUE, "Plot.Fill/Pt. Color"=w356) -> (error out=w355:errorcluster)  [unwired: 2 in, 1 out]
                n233 = Bundle(FALSE) -> (w353:cluster{bool})  [unwired: 1 in]
                n234 = Bundle(TRUE) -> (w354:cluster{bool})  [unwired: 1 in]
                n235 = Build Array(w353, w354) -> (w350:cluster{bool}[])
              }
              n236 = local write "Couleurs"(w349) -> ()
              n237 = local write "Y1/Y2"(w342) -> ()
              n238 = property on="Courbe" class="GraphXY (strict)"(error in=w344, "ActYScl"=0 ("Échelle active des Y"), "YScale.Visible"=FALSE ("Échelle des Y.Visible"), "ActYScl"=1 ("Échelle active des Y"), "YScale.Visible"=TRUE ("Échelle des Y.Visible")) -> (error out=w343:errorcluster)  [unwired: 1 in, 1 out]
              n239 = call <vilib>:"Clear Errors.vi"("error in (no error)"=w343) -> ()  [unwired: 5 in, 2 out]
            }
            event "Tout OFF": Value Change {
              n240 = event-data() -> ()  [unwired: 1 in, 5 out]
              n241 = local read "Couleurs"() -> (w369:u32[])
              n242 = for {
                tunnel: w369 -> [_] mode=indexing
                tunnel: [u32 16777216 ("nouvel élément/sous-tableau")] -> w368 mode=indexing
                tunnel: [w375] -> w363
                tunnel: [w370] -> w361 mode=indexing
                i -> [w377]
                n243 = Bundle(FALSE) -> (w373:cluster{bool})  [unwired: 1 in]
                n244 = Bundle(FALSE) -> (w374:cluster{bool})  [unwired: 1 in]
                n245 = property on="Courbe" class="GraphXY (strict)"("Active Plot"=w377, "Plot.Visible?"=FALSE) -> (error out=w375:errorcluster)  [unwired: 2 in, 1 out]
                n246 = Build Array(w373, w374) -> (w370:cluster{bool}[])
              }
              n247 = local write "Couleurs"(w368) -> ()
              n248 = local write "Y1/Y2"(w361) -> ()
              n249 = property on="Courbe" class="GraphXY (strict)"(error in=w363, "ActYScl"=0 ("Échelle active des Y"), "YScale.Visible"=FALSE ("Échelle des Y.Visible"), "ActYScl"=1 ("Échelle active des Y"), "YScale.Visible"=FALSE ("Échelle des Y.Visible")) -> (error out=w362:errorcluster)  [unwired: 1 in, 1 out]
              n250 = call <vilib>:"Clear Errors.vi"("error in (no error)"=w362) -> ()  [unwired: 5 in, 2 out]
            }
            event "Calcul Pente": Value Change {
              n251 = event-data() -> ("NewVal"=w379:bool)  [unwired: 1 in, 5 out]
              n252 = property on="Courbe" class="GraphXY (strict)"() -> ("XScale.Maximum"=w387:dbl, "XScale.Minimum"=w383:dbl)  [unwired: 2 in, 2 out]
              n253 = property on="Pente" class="NumNb (strict)"("Visible"=w379) -> ()  [unwired: 2 in, 2 out]
              n254 = property on="Unités par" class="MDér (strict)"("Visible"=w379) -> ()  [unwired: 2 in, 2 out]
              n255 = property on="Capteur" class="MDér (strict)"("Visible"=w379) -> ()  [unwired: 2 in, 2 out]
              n256 = property on="Courbe" class="GraphXY (strict)"("Active Cursor"=u32 0 ("Curseur actif"), "Cursor.Visible"=w379, "Active Cursor"=u32 1 ("Curseur actif"), "Cursor.Visible"=w379) -> ()  [unwired: 2 in, 2 out]
              n257 = Subtract(x=w387, y=w383) -> (x-y=w386:dbl)
              n258 = Divide(x=w386, y=2.0) -> (x/y=w384:dbl)
              n259 = Add(x=w384, y=w383) -> (x+y=w382:dbl)
              n260 = property on="Courbe" class="GraphXY (strict)"("Active Cursor"=u32 0 ("Curseur actif"), "Cursor.Cursor X"=w382, "Active Cursor"=u32 1 ("Curseur actif"), "Cursor.Cursor X"=w382) -> ()  [unwired: 2 in, 2 out]
            }
            event "Unités par", "Capteur": Value Change; "Courbe": Cursor Release {
              n261 = event-data() -> ()  [unwired: 1 in, 4 out]
              n262 = property on="Courbe" class="GraphXY (strict)"("Active Cursor"=u32 0 ("Curseur actif"), "Cursor.Cursor Plot"="Capteur", "Active Cursor"=u32 1 ("Curseur actif"), "Cursor.Cursor Plot"="Capteur") -> ("Cursor.Cursor X"=w391:dbl, "Cursor.Cursor Y"=w392:dbl, "Cursor.Cursor X"=w393:dbl, "Cursor.Cursor Y"=w394:dbl)  [unwired: 2 in, 2 out]
              n263 = Max & Min(x=w392, y=w394) -> (max(x,y)=w403:dbl, min(x,y)=w402:dbl)
              n264 = Max & Min(x=w391, y=w393) -> (max(x,y)=w401:dbl, min(x,y)=w400:dbl)
              n265 = Subtract(x=w403, y=w402) -> (x-y=w399:dbl)
              n266 = Subtract(x=w401, y=w400) -> (x-y=w398:dbl)
              n267 = Divide(x=w399, y=w398) -> (x/y=w397:dbl)
              n268 = case shown="2" "Unités par" {
                tunnel: w397 -> [w406 w407 w411]
                tunnel: [w406 w408 w410] -> w396
                frame 0, Default {
                  # "seconde"
                }
                frame 1 {
                  # "minute"
                  n269 = Multiply(x=w407, y=60.0) -> (x*y=w408:dbl)
                }
                frame 2 {
                  # "heure"
                  n270 = Multiply(x=w411, y=3600.0) -> (x*y=w410:dbl)
                }
              }
              "Pente" <- w396
            }
            event "SORTIR VISU": Value Change {
              n271 = event-data() -> ("NewVal"=w413:bool)  [unwired: 1 in, 4 out]
              n272 = case shown="Vrai" w413 {
                frame False {
                }
                frame True {
                  n273 = call "Boite Dialogue 2 boutons.vi"("bouton droit visible ?"=TRUE, "Texte bouton droit"="OUI" ("Texte bouton gauche"), "Texte bouton gauche"="NON" ("Texte bouton droit"), "Message"="Vous avez demandé de sortir de la visualisation graphique.\nA la prochaine ouverture, le graphe sera réinitialisé\n(il ne comportera que le dernier fichier)\nVoulez-vous continuer ?") -> ("Bouton droit ?"=→"SORTIE VISU":bool)
                  n274 = local write "SORTIR VISU"(FALSE ("SORTIR VISU")) -> ()
                }
              }
            }
          }
          n275 = global read "Variable glob generale.vi" "Lancement"() -> (w153:bool)
          n276 = local read "SORTIE VISU"() -> (w154:bool)
          n277 = Not(x=w153) -> (.not. x?=w152:bool)
          n278 = Or(x=w154, y=w152) -> (x .or. y?=w155:bool)
        }
        n279 = Not Equal?(x=w149, y="") -> (x != y?=w147:bool)
        n280 = local read "nb capt"() -> (w145:i32)
        n281 = property on="commentaire" class="Ch"("Visible"=w147) -> ()  [unwired: 2 in, 2 out]
        n282 = while {
          shift-right: [w437] -> _
          shift-left: w151 -> [w439]
          shift-right: [w436] -> _
          shift-left: w150 -> [w438]
          shift-right: [w435] -> _
          shift-left: _ -> [w434]
          tunnel: w145 -> [w433]
          tunnel: w146 -> [w421]
          stop <- w425 stop-if-true
          # "données"
          # "temps"
          n283 = feedback #1(w421) -> (w422:i64)
          n284 = call "Nouvelles donnees.vi"("Nb Capteurs"=w433, "offset entrée (en octets) (0)"=w422) -> ("Nouvelles données"=w420:string[], "Nouveau temps"=w435:dbl, "Chemin du fichier local :"=→"Chemin du fichier local":path, "offset sortie (en octets)"=w423:i64)
          "Données" <- w420
          n285 = feedback-in #1(w423) -> ()
          n286 = Equal?(x=w434, y=w435) -> (x = y?=w431:bool)
          n287 = Equal To 0?(x=w435) -> (x = 0?=w430:bool)
          n288 = Or(x=w431, y=w430) -> (x .or. y?=w429:bool)
          n289 = case shown="Faux" w429 {
            tunnel: w439 -> [w447 w474]
            tunnel: w438 -> [w454 w473]
            tunnel: [w458 w474] -> w437
            tunnel: [w451 w473] -> w436
            tunnel: w420 -> [w449 _]
            tunnel: w435 -> [w453 _]
            frame False {
              # "12h pour 28 capteurs\ntoutes les 1s"
              n290 = Array Size(array=w447) -> (size(s)=w446:i32[])
              n291 = Index Array(array=w446, index #1=0 ("indice"), index #2=1 ("indice")) -> (element #1=w442:i32, element #2=w443:i32)
              n292 = Multiply(x=w442, y=w443) -> (x*y=w441:i32)
              n293 = Fract/Exp String To Number(string=w449) -> (number=w450:dbl[])  [unwired: 3 in, 1 out]
              n294 = Greater?(x=w441, y=1200000) -> (0:w448:bool)
              n295 = case shown="Vrai" w448 {
                tunnel: [w459 w461] -> w456
                tunnel: [w460 w462] -> w455
                tunnel: w454 -> [w459 w468]
                tunnel: w447 -> [w460 w465]
                frame False {
                }
                frame True {
                  n296 = Delete From Array(array=w468, length=1 ("longueur"), index=0 ("indice")) -> (array with subset deleted=w461:dbl[])  [unwired: 1 out]
                  n297 = Delete From Array(array=w465, length=1 ("longueur"), index (row)=0 ("indice (ligne)")) -> (array with subset deleted=w462:dbl[][])  [unwired: 1 in, 1 out]
                }
              }
              n298 = Build Array (concatenate)(w455, w450) -> (w458:dbl[][])
              n299 = Build Array (concatenate)(w456, w453) -> (w451:dbl[])
              n300 = Transpose 2D Array(2D array=w458) -> (transposed array=w452:dbl[][])
              n301 = for {
                tunnel: w452 -> [w470] mode=indexing
                tunnel: w451 -> [w471]
                tunnel: [w472] -> w457 mode=indexing
                n302 = Bundle(w471, w470) -> (w472:cluster{dbl[], dbl[]})  [unwired: 1 in]
                n303 = Wait (ms)(milliseconds to wait=u32 10 ("attente (ms)")) -> ()  [unwired: 1 out]
              }
              "Courbe" <- w457
            }
            frame True {
              # "pas de nouvelles données\nou ligne vide => temps = 0"
            }
          }
          n304 = Wait Until Next ms Multiple(millisecond multiple=u32 1000 ("n millisecondes")) -> ()  [unwired: 1 out]
          n305 = local read "SORTIE VISU"() -> (w427:bool)
          n306 = global read "Variable glob generale.vi" "Lancement"() -> (w426:bool)
          n307 = Not(x=w426) -> (.not. x?=w424:bool)
          n308 = Or(x=w427, y=w424) -> (x .or. y?=w425:bool)
        }
      }
      frame "fin" {
        # "enregistrement des couleurs"
        n309 = global read "Variable glob generale.vi" "Couleurs"() -> (w475:u32[])
        n310 = disable-structure shown="Activé" {
          disable-tunnel: [w493 w501] -> w482
          disable-tunnel: w475 -> [w492 w502]
          frame Disabled {
            n311 = Array To Spreadsheet String(delimiter (Tab)=";" ("séparateur (Tabulation)"), array=w492, 3:"%d" ("chaîne de format")) -> (spreadsheet string=w494:string)
            n312 = String Length(string=w494) -> (length=w498:i32)
            n313 = Subtract(x=w498, y=2) -> (x-y=w496:i32)
            n314 = String Subset(string=w494, offset (0)=0, length (rest)=w496) -> (substring=w493:string)
          }
          frame Enabled {
            n315 = Number To Fractional String(number=w502, precision (6)=i16 2 ("précision (6)")) -> (F-format string=w504:string[])  [unwired: 2 in]
            n316 = call "Tableau en chaine.vi"("Tableau 1D"=w504) -> ("Chaîne"=w501:string)  [unwired: 1 in, 1 out]
          }
        }
        n317 = disable-structure shown="Activé" {
          frame Enabled {
            n318 = local read "référence en sortie"() -> (w508:refnum<vi>)
            n319 = invoke class="VI" method="FA.Fermer"(reference=w508) -> (reference out=w506:refnum<vi>, error out=w507:errorcluster)  [unwired: 2 in, 1 out]
            n320 = Close Reference(reference=w506, error in (no error)=w507) -> (error out=w505:errorcluster)
            n321 = call <vilib>:"Clear Errors.vi"("error in (no error)"=w505) -> ()  [unwired: 5 in, 2 out]
          }
          frame Disabled {
          }
        }
        n322 = Request Deallocation(TRUE ("flag")) -> ()
        n323 = Build Path(base path=path "C:/LABVIEW/PRES+TEMP+REG dernière version/Configurations", name or relative path="config acqui.ini" ("nom ou chemin relatif")) -> (appended path=w490:path)
        n324 = call <vilib>:"Open Config Data.vi"("create file if necessary (T)"=TRUE ("create file if necessary? (T)"), "configuration file path"=w490) -> ("error out"=w488:errorcluster, "refnum"=w487:T12)  [unwired: 7 in, 1 out]
        n325 = call-poly <vilib>:"Write Key.vi"("section"="GENERAL", "error in (no error)"=w488, "value"=w482, "key"="COULEURS", "refnum"=w487) -> ("error out"=w483:errorcluster, "refnum out"=w484:T12)  [unwired: 4 in, 1 out]
        n326 = call <vilib>:"Close Config Data.vi"("error in (no error)"=w483, "refnum"=w484) -> ("error out"=w480:errorcluster)  [unwired: 8 in, 1 out]
        n327 = call <vilib>:"Clear Errors.vi"("error in (no error)"=w480) -> ()  [unwired: 5 in, 2 out]
        n328 = global write "Variable glob generale.vi" "Visu en cours"(FALSE ("Visu en cours")) -> ()
      }
    }
  }
